vi "configure eipt.vi"(8 "error in":errorcluster, 10 "tag definition in":T2, 11 "EthernetIP configuration":refnum<class "EIP Tags Configuration.lvclass">) -> (0 "error out":errorcluster, 1 "success":bool, 2 "tag definition out":T2, 5 "changed":bool)   [LabVIEW 2013, in "EIP Tags editor node.lvclass"]
uses:
  EIP Tags editor node.lvclass
  configuration/EIP Tags Configuration.lvclass
  configuration/eip tag types.ctl
  configuration/eip tag definition.ctl
panel:
  in  "Tag Name":string
  in  "Network path (ip,backplane port, logix slot)":string
  in  "Number of Elements":u32
  in  "Tag Type":T1
  in  "cancel":bool
  in  "ok":bool
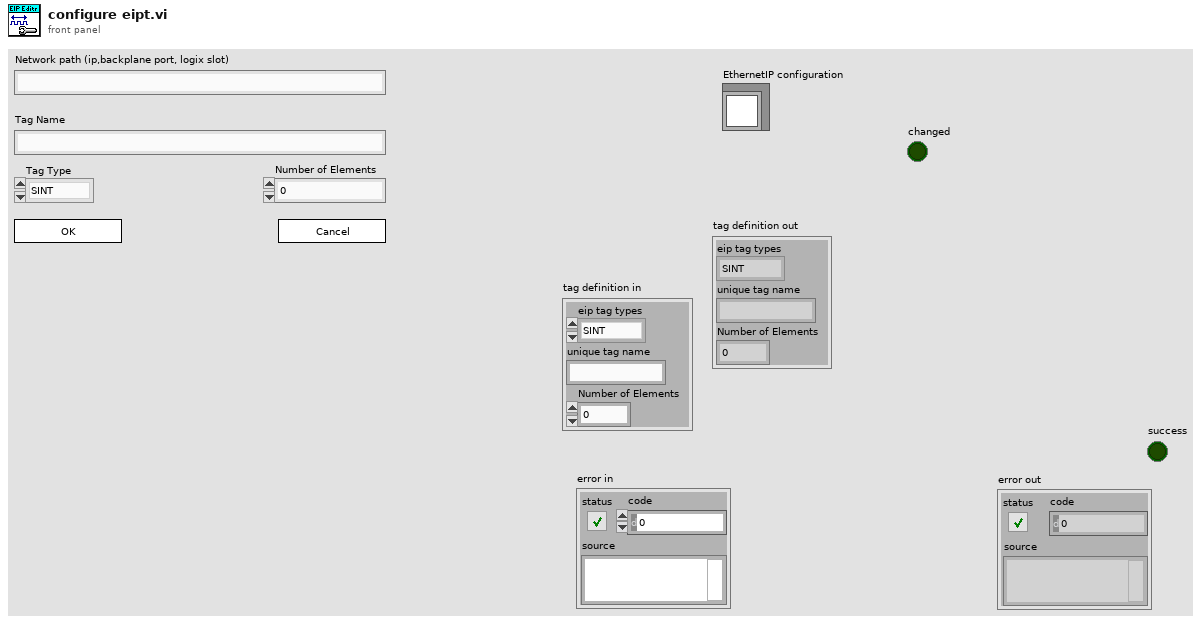
[diagram p1: front panel]
types:
  T1 = typedef "EIP Tags Configuration.lvclass/eip tag types.ctl" = enum16{"SINT", "INT", "DINT", "REAL", "BOOL", "STRING"}
  T2 = typedef "EIP Tags Configuration.lvclass/eip tag definition.ctl" = cluster{"eip tag types":T1, "unique tag name":string, "Number of Elements":u32}
  T3 = enum32{"Invalid", "Standard", "Closed", "Hidden", "Minimized", "Maximized"}
  T4 = enum32{"Invalid", "Default", "Floating", "Floating/Auto-Hide", "Modal"}
  T5 = enum8{"Enabled", "Disabled", "Disabled and Grayed Out"}
  T6 = enum32{"invalid app kind", "Development System", "Run Time System", "Student Edition", "Embedded LabVIEW", "Evaluation", "Custom"}
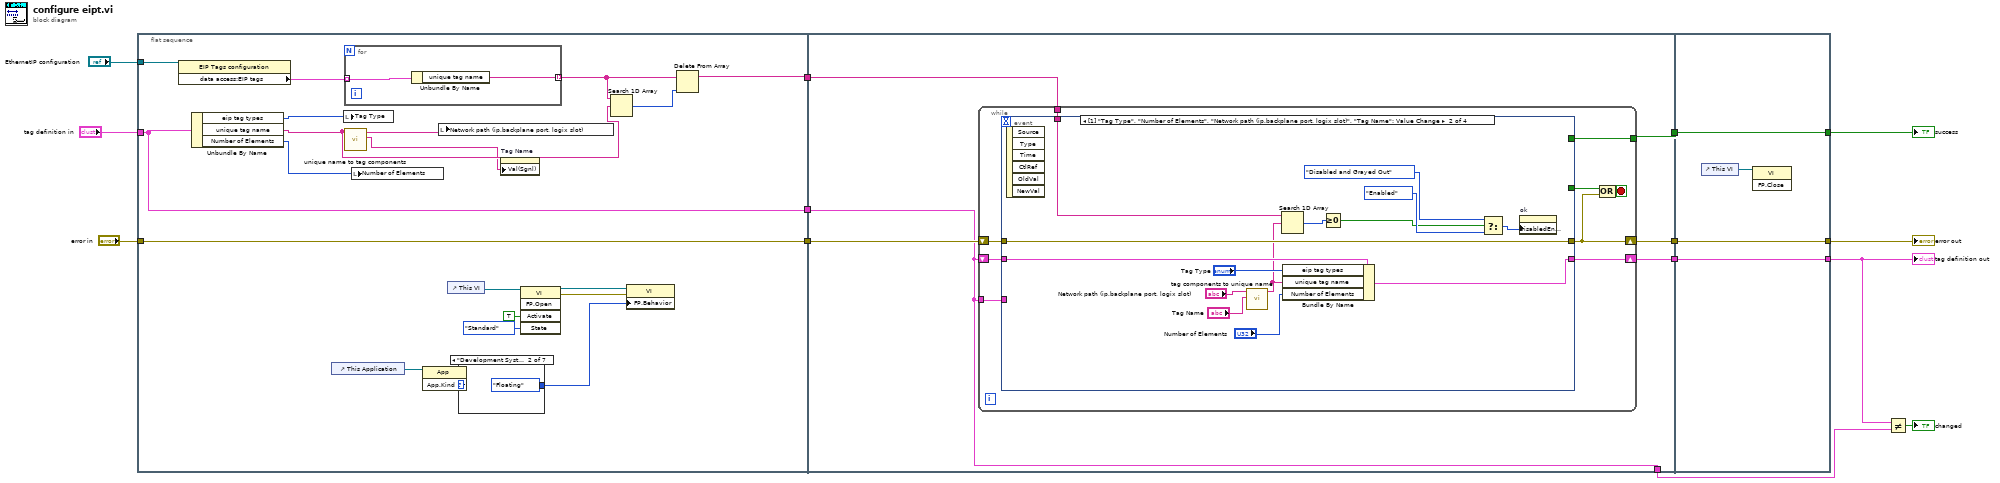
[diagram p0: block diagram]
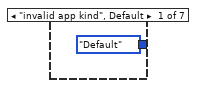
[diagram p2: hidden frame]
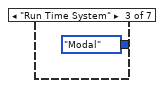
[diagram p3: hidden frame]
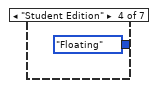
[diagram p4: hidden frame]
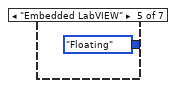
[diagram p5: hidden frame]
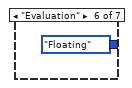
[diagram p6: hidden frame]
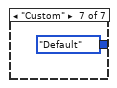
[diagram p7: hidden frame]
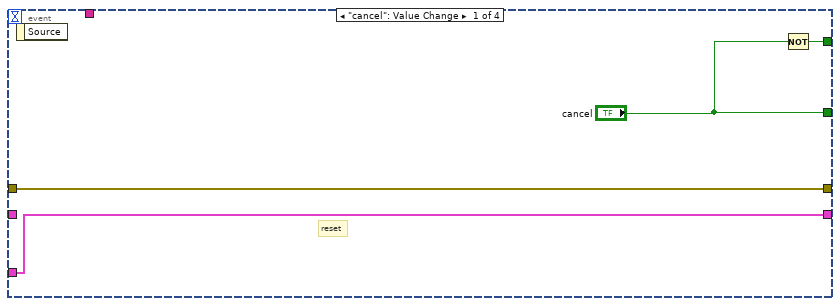
[diagram p8: hidden frame]
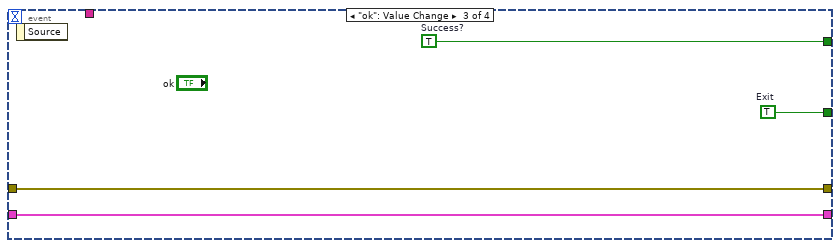
[diagram p9: hidden frame]
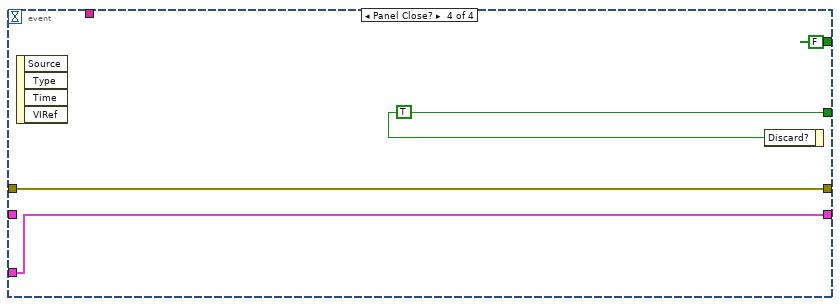
[diagram p10: hidden frame]
diagram:
  n1 = flat-sequence {
    tunnel: "error in" -> [w26]
    tunnel: "EthernetIP configuration" -> [w21]
    tunnel: "tag definition in" -> [w25]
    tunnel: [w26] -> w5
    tunnel: [w25] -> w4
    tunnel: [w16] -> w1
    tunnel: [w49] -> w10
    tunnel: [w48] -> w9
    tunnel: [w47] -> w8
    tunnel: w5 -> [w46]
    tunnel: w4 -> [w45]
    tunnel: [w45] -> w3
    tunnel: w1 -> [w44]
    tunnel: [w86] -> w2
    tunnel: [w87] -> w12
    tunnel: [w88] -> w13
    tunnel: w10 -> [w88]
    tunnel: w9 -> [w87]
    tunnel: w8 -> [w86]
    frame #0 {
      n2 = property class="EIP Tags configuration"(reference=w21) -> ("data access:EIP tags"=w20:T2[])  [unwired: 1 in, 2 out]
      n3 = Unbundle By Name(w25) -> ("eip tag types"=w22:T1, "unique tag name"=w19:string, "Number of Elements"=w23:u32)
      n4 = control-ref of="This Application"() -> (w29:refnum<vi>)
      n5 = local write "Tag Type"(w22) -> ()
      n6 = for {
        tunnel: w20 -> [w36] mode=indexing
        tunnel: [w35] -> w18 mode=indexing
        n7 = Unbundle By Name(w36) -> ("unique tag name"=w35:string)
      }
      n8 = call "unique name to tag components.vi"("unique name"=w19) -> ("Tag Name"=w15:string, "Network Path"=w24:string)  [unwired: 9 in]
      n9 = local write "Number of Elements"(w23) -> ()
      n10 = property class="App"(reference=w29) -> ("App.Kind"=w28:T6)  [unwired: 1 in, 2 out]
      n11 = local write "Network path (ip,backplane port, logix slot)"(w24) -> ()
      n12 = control-ref of="This VI"() -> (w30:refnum<vi>)
      n13 = case shown="\"Development System\"" w28 {
        tunnel: [T4."Default" ("Front Panel Window:Behavior") T4."Floating" ("Front Panel Window:Behavior") T4."Modal" ("Front Panel Window:Behavior") T4."Floating" ("Front Panel Window:Behavior") T4."Floating" ("Front Panel Window:Behavior") T4."Floating" ("Front Panel Window:Behavior") T4."Default" ("Front Panel Window:Behavior")] -> w27
        frame "invalid app kind", Default {
        }
        frame "Development System" {
        }
        frame "Run Time System" {
        }
        frame "Student Edition" {
        }
        frame "Embedded LabVIEW" {
        }
        frame "Evaluation" {
        }
        frame "Custom" {
        }
      }
      n14 = property on="Tag Name" class="Str"("Val(Sgnl)"=w15) -> ()  [unwired: 2 in, 2 out]
      n15 = invoke class="VI" method="FP.Open"(reference=w30, "Activate"=TRUE ("Activate?"), "State"=T3."Standard") -> (reference out=w33:refnum<vi>, error out=w34:errorcluster)  [unwired: 2 in, 3 out]
      n16 = Search 1D Array(1D array=w18, element=w19) -> (index of element=w17:i32)  [unwired: 1 in]
      n17 = property class="VI"(reference=w33, error in=w34, "FP.Behavior"=w27) -> ()  [unwired: 2 out]
      n18 = Delete From Array(array=w18, index=w17) -> (array with subset deleted=w16:string[])  [unwired: 1 in, 1 out]
    }
    frame #1 {
      n19 = while {
        shift-right: [w53] -> w48
        shift-left: w46 -> [w58]
        tunnel: [w57] -> w49
        shift-right: [w51] -> w47
        shift-left: w45 -> [w54]
        tunnel: w45 -> [w52]
        tunnel: w44 -> [w50]
        stop <- w55 stop-if-true
        n20 = event shown="[1] \"Tag Type\", \"Number of Elements\", \"Network path (ip,backplane port, logix slot)\", \"Tag Name\": Value Change" {
          selector: _ -> [_ _ _ _]
          dyn-events: _ -> [_ _ _ _]
          timeout: _ -> [_ _ _ _]
          tunnel: w58 -> [w62 w76 w80 w84]
          tunnel: [w62 w76 w80 w84] -> w53
          tunnel: [w61 _ w77 FALSE] -> w57
          tunnel: ["cancel" _ w78 w82] -> w56
          tunnel: w54 -> [_ w75 w79 _]
          tunnel: [w59 w74 w79 w81] -> w51
          tunnel: w52 -> [w59 _ _ w81]
          tunnel: w50 -> [_ w68 _ _]
          event "cancel": Value Change {
            # "reset"
            n21 = event-data() -> ()  [unwired: 1 in, 1 out]
            n22 = Not(x="cancel") -> (.not. x?=w61:bool)
          }
          event "Number of Elements", "Network path (ip,backplane port, logix slot)", "Tag Name": Value Change {
            n23 = event-data() -> ()  [unwired: 1 in, 6 out]
            n24 = call "tag components to unique name.vi"("Tag Name"="Tag Name", "Network Path"="Network path (ip,backplane port, logix slot)") -> ("unique name"=w69:string)  [unwired: 9 in]
            n25 = Search 1D Array(1D array=w68, element=w69) -> (index of element=w67:i32)  [unwired: 1 in]
            n26 = Bundle By Name(cluster=w75, "eip tag types"="Tag Type", "unique tag name"=w69, "Number of Elements"="Number of Elements") -> (w74:T2)
            n27 = Greater Or Equal To 0?(x=w67) -> (x >= 0?=w63:bool)
            n28 = Select(t=T5."Disabled and Grayed Out" ("Disabled"), s=w63, f=T5."Enabled" ("Disabled")) -> (s? t:f=w65:T5)
            n29 = property on="ok" class="Bool"("DisabledEnum"=w65) -> ()  [unwired: 2 in, 2 out]
          }
          event "ok": Value Change {
            w77 = TRUE  # Success?
            w78 = TRUE  # Exit
            n30 = event-data() -> ()  [unwired: 1 in, 1 out]
          }
          event Panel Close? {
            w82 = TRUE ("cancel")
            n31 = event-data() -> ()  [unwired: 1 in, 4 out]
            n32 = event-data("Discard?"=w82) -> ()  [unwired: 1 in, 1 out]
          }
        }
        n33 = Compound Arithmetic op=OR(w56, w53) -> (w55:bool)
      }
    }
    frame #2 {
      n34 = control-ref of="This VI"() -> (w85:refnum<vi>)
      n35 = invoke class="VI" method="FP.Close"(reference=w85) -> ()  [unwired: 2 in, 3 out]
    }
  }
  n36 = Not Equal?(x=w2, y=w3) -> (x != y?=→"changed":bool)
  "error out" <- w12
  "success" <- w13
  "tag definition out" <- w2
